vi "Set LED.vi"(8 "error in (no error)":errorcluster, 10 "LED State":bool, 11 "AS7431 Light Spectrum in":refnum<class "AS7431 11 Ch Light Spectrum Sensor.lvclass">) -> (0 "error out":errorcluster, 3 "AS7431 Light Spectrum out":refnum<class "AS7431 11 Ch Light Spectrum Sensor.lvclass">)   [LabVIEW 2020, in "CTI-Peripheral.lvlib" / "AS7431 11 Ch Light Spectrum Sensor.lvclass"]
uses:
  AS7431 11 Ch Light Spectrum Sensor.lvclass
  AS7431 11 Ch Light Spectrum Sensor.lvclass/AS7431 11 Ch Light Spectrum Sensor.ctl
  CTI/I2C Connection/I2C Connection.lvclass/I2C Connection.ctl
  CTI/Session/I2C Write Data.vi
  CTI/Session/I2C Read Data.vi
  CTI/I2C Connection/I2C Connection.lvclass
panel:
  out "Data":string
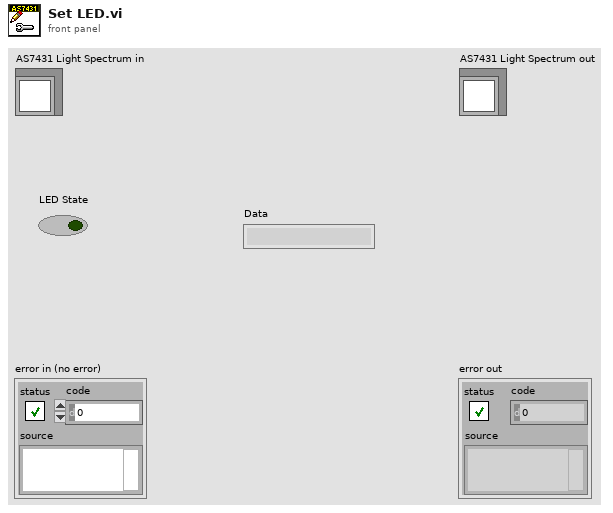
[diagram p1: front panel]
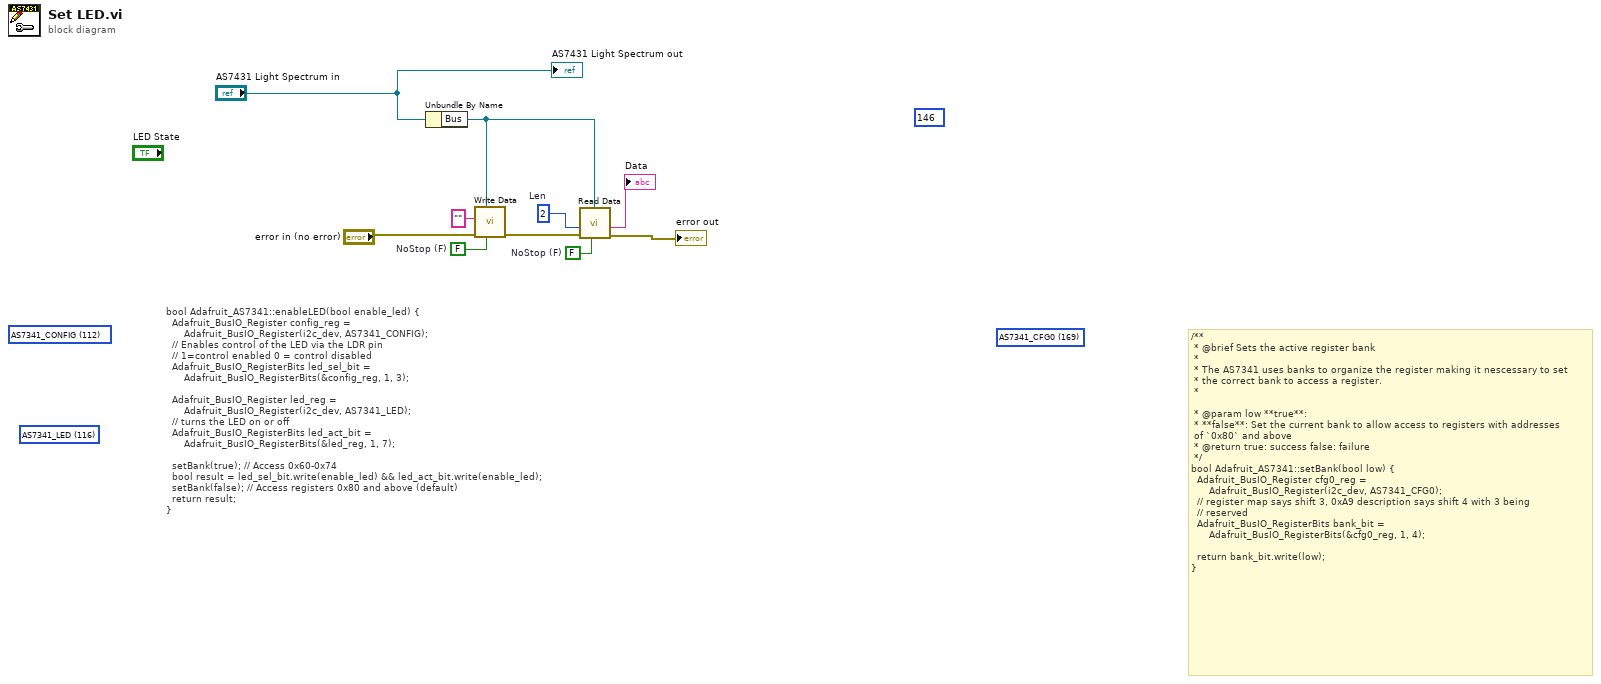
[diagram p0: block diagram]
diagram:
  (unwired) 146
  (unwired) u16 169 items=["AS7341_I2CADDR_DEFAULT"=57, "AS7341_CHIP_ID"=9, "AS7341_WHOAMI"=146, "AS7341_CONFIG"=112, "AS7341_GPIO"=115, "AS7341_LED"=116, "AS7341_ENABLE"=128, "AS7341_ATIME"=129, "AS7341_SP_LOW_TH_L"=132, "AS7341_SP_LOW_TH_H"=133, "AS7341_SP_HIGH_TH_L"=134, "AS7341_SP_HIGH_TH_H"=135, "AS7341_STATUS"=147, "AS7341_ASTATUS_"=148, "AS7341_CH0_DATA_L"=149, "AS7341_CH0_DATA_H"=150, "AS7341_CH1_DATA_L"=151, "AS7341_CH1_DATA_H"=152, "AS7341_CH2_DATA_L"=153, "AS7341_CH2_DATA_H"=154, "AS7341_CH3_DATA_L"=155, "AS7341_CH3_DATA_H"=156, "AS7341_CH4_DATA_L"=157, "AS7341_CH4_DATA_H"=158, "AS7341_CH5_DATA_L"=159, "AS7341_CH5_DATA_H"=160, "AS7341_STATUS2"=163, "AS7341_STATUS3"=164, "AS7341_CFG0"=169, "AS7341_CFG1"=170, "AS7341_CFG6"=175, "AS7341_CFG9"=178, "AS7341_CFG12"=181, "AS7341_PERS"=189, "AS7341_GPIO2"=190, "AS7341_ASTEP_L"=202, "AS7341_ASTEP_H"=203, "AS7341_FD_TIME1"=216, "AS7341_FD_TIME2"=218, "AS7341_FD_STATUS"=219, "AS7341_INTENAB"=249, "AS7341_CONTROL"=250] ("Registers")
  (unwired) u16 116 items=["AS7341_I2CADDR_DEFAULT"=57, "AS7341_CHIP_ID"=9, "AS7341_WHOAMI"=146, "AS7341_CONFIG"=112, "AS7341_GPIO"=115, "AS7341_LED"=116, "AS7341_ENABLE"=128, "AS7341_ATIME"=129, "AS7341_SP_LOW_TH_L"=132, "AS7341_SP_LOW_TH_H"=133, "AS7341_SP_HIGH_TH_L"=134, "AS7341_SP_HIGH_TH_H"=135, "AS7341_STATUS"=147, "AS7341_ASTATUS_"=148, "AS7341_CH0_DATA_L"=149, "AS7341_CH0_DATA_H"=150, "AS7341_CH1_DATA_L"=151, "AS7341_CH1_DATA_H"=152, "AS7341_CH2_DATA_L"=153, "AS7341_CH2_DATA_H"=154, "AS7341_CH3_DATA_L"=155, "AS7341_CH3_DATA_H"=156, "AS7341_CH4_DATA_L"=157, "AS7341_CH4_DATA_H"=158, "AS7341_CH5_DATA_L"=159, "AS7341_CH5_DATA_H"=160, "AS7341_STATUS2"=163, "AS7341_STATUS3"=164, "AS7341_CFG0"=169, "AS7341_CFG1"=170, "AS7341_CFG6"=175, "AS7341_CFG9"=178, "AS7341_CFG12"=181, "AS7341_PERS"=189, "AS7341_GPIO2"=190, "AS7341_ASTEP_L"=202, "AS7341_ASTEP_H"=203, "AS7341_FD_TIME1"=216, "AS7341_FD_TIME2"=218, "AS7341_FD_STATUS"=219, "AS7341_INTENAB"=249, "AS7341_CONTROL"=250] ("Registers")
  (unwired) u16 112 items=["AS7341_I2CADDR_DEFAULT"=57, "AS7341_CHIP_ID"=9, "AS7341_WHOAMI"=146, "AS7341_CONFIG"=112, "AS7341_GPIO"=115, "AS7341_LED"=116, "AS7341_ENABLE"=128, "AS7341_ATIME"=129, "AS7341_SP_LOW_TH_L"=132, "AS7341_SP_LOW_TH_H"=133, "AS7341_SP_HIGH_TH_L"=134, "AS7341_SP_HIGH_TH_H"=135, "AS7341_STATUS"=147, "AS7341_ASTATUS_"=148, "AS7341_CH0_DATA_L"=149, "AS7341_CH0_DATA_H"=150, "AS7341_CH1_DATA_L"=151, "AS7341_CH1_DATA_H"=152, "AS7341_CH2_DATA_L"=153, "AS7341_CH2_DATA_H"=154, "AS7341_CH3_DATA_L"=155, "AS7341_CH3_DATA_H"=156, "AS7341_CH4_DATA_L"=157, "AS7341_CH4_DATA_H"=158, "AS7341_CH5_DATA_L"=159, "AS7341_CH5_DATA_H"=160, "AS7341_STATUS2"=163, "AS7341_STATUS3"=164, "AS7341_CFG0"=169, "AS7341_CFG1"=170, "AS7341_CFG6"=175, "AS7341_CFG9"=178, "AS7341_CFG12"=181, "AS7341_PERS"=189, "AS7341_GPIO2"=190, "AS7341_ASTEP_L"=202, "AS7341_ASTEP_H"=203, "AS7341_FD_TIME1"=216, "AS7341_FD_TIME2"=218, "AS7341_FD_STATUS"=219, "AS7341_INTENAB"=249, "AS7341_CONTROL"=250] ("Registers")
  w7 = FALSE  # NoStop (F)
  w8 = u8 2  # Len
  w9 = FALSE  # NoStop (F)
  # "/**\n * @brief Sets the active register bank\n *\n * The AS7341 uses banks to organize the register making it nescessary to set\n * the correct bank to access a register.\n *\n\n * @param low **true**:\n * **false**: Set the current bank to allow access to registers with addresses\n of `0x80` and above\n * @return true: success false: failure\n */\nbool Adafruit_AS7341::setBank(bool low) {\n  Adafruit_BusIO_Register cfg0_reg =\n      Adafruit_BusIO_Register(i2c_dev, AS7341_CFG0);\n  // register map says shift 3, 0xA9 description says shift 4 with 3 being\n  // reserved\n  Adafruit_BusIO_RegisterBits bank_bit =\n      Adafruit_BusIO_RegisterBits(&cfg0_reg, 1, 4);\n\n  return bank_bit.write(low);\n}"
  # "bool Adafruit_AS7341::enableLED(bool enable_led) {\n  Adafruit_BusIO_Register config_reg =\n      Adafruit_BusIO_Register(i2c_dev, AS7341_CONFIG);\n  // Enables control of the LED via the LDR pin\n  // 1=control enabled 0 = control disabled\n  Adafruit_BusIO_RegisterBits led_sel_bit =\n      Adafruit_BusIO_RegisterBits(&config_reg, 1, 3);\n\n  Adafruit_BusIO_Register led_reg =\n      Adafruit_BusIO_Register(i2c_dev, AS7341_LED);\n  // turns the LED on or off\n  Adafruit_BusIO_RegisterBits led_act_bit =\n      Adafruit_BusIO_RegisterBits(&led_reg, 1, 7);\n\n  setBank(true); // Access 0x60-0x74\n  bool result = led_sel_bit.write(enable_led) && led_act_bit.write(enable_led);\n  setBank(false); // Access registers 0x80 and above (default)\n  return result;\n}"
  n1 = Unbundle By Name("AS7431 Light Spectrum in") -> ("Bus"=w6:refnum<class "I2C Connection.lvclass">)
  n2 = call "Write Data.vi"("NoStop (F)"=w9, "I2C Connection"=w6, "error in (no error)"="error in (no error)", "Data"="") -> ("error out"=w5:errorcluster)  [unwired: 7 in]
  n3 = call "Read Data.vi"("NoStop (F)"=w7, "I2C Connection"=w6, "error in (no error)"=w5, "Len"=w8) -> ("error out"=→"error out":errorcluster, "Data"=→"Data":string)  [unwired: 6 in]
  "AS7431 Light Spectrum out" <- "AS7431 Light Spectrum in"
